vi "Ecrire Prog MODBUS EPC.vi"(0 "Adresse rég":u8 caption="Adresse régulateur", 1 "Programme":cluster{"chaîne o":string, "Value":dbl}[][](array[cluster]), 2 "N° prog":u16 caption="Numéro de programme", 3 "error in":errorcluster caption="error IO", 4 "Port COM run 1 REG":refnum<visa-resource-name>) -> (6 "error out":errorcluster caption="error IO")   [LabVIEW 2022 SP3]
uses:
  Variables globales/Variables glob EUROTHERM.vi
panel:
  out "error IO":errorcluster caption="error par segment"
  out "unité rampe":u16
  out "unité palier":u16
  out "Numéro segment":u16
  out "adr type fin":u64
  out "Nom rég":string caption="Nom régulateur"
  # "écrire un programme"
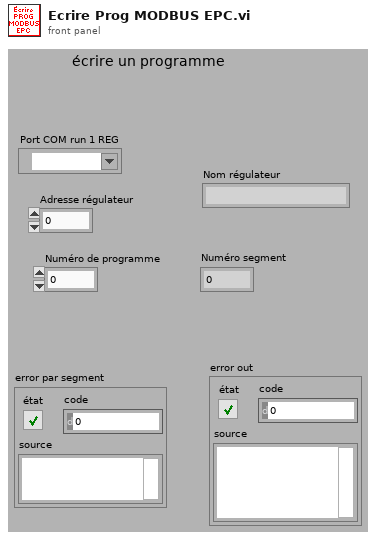
[diagram p1: front panel]
types:
  T1 = typedef "Semaphore RefNum" = refnum<k1>
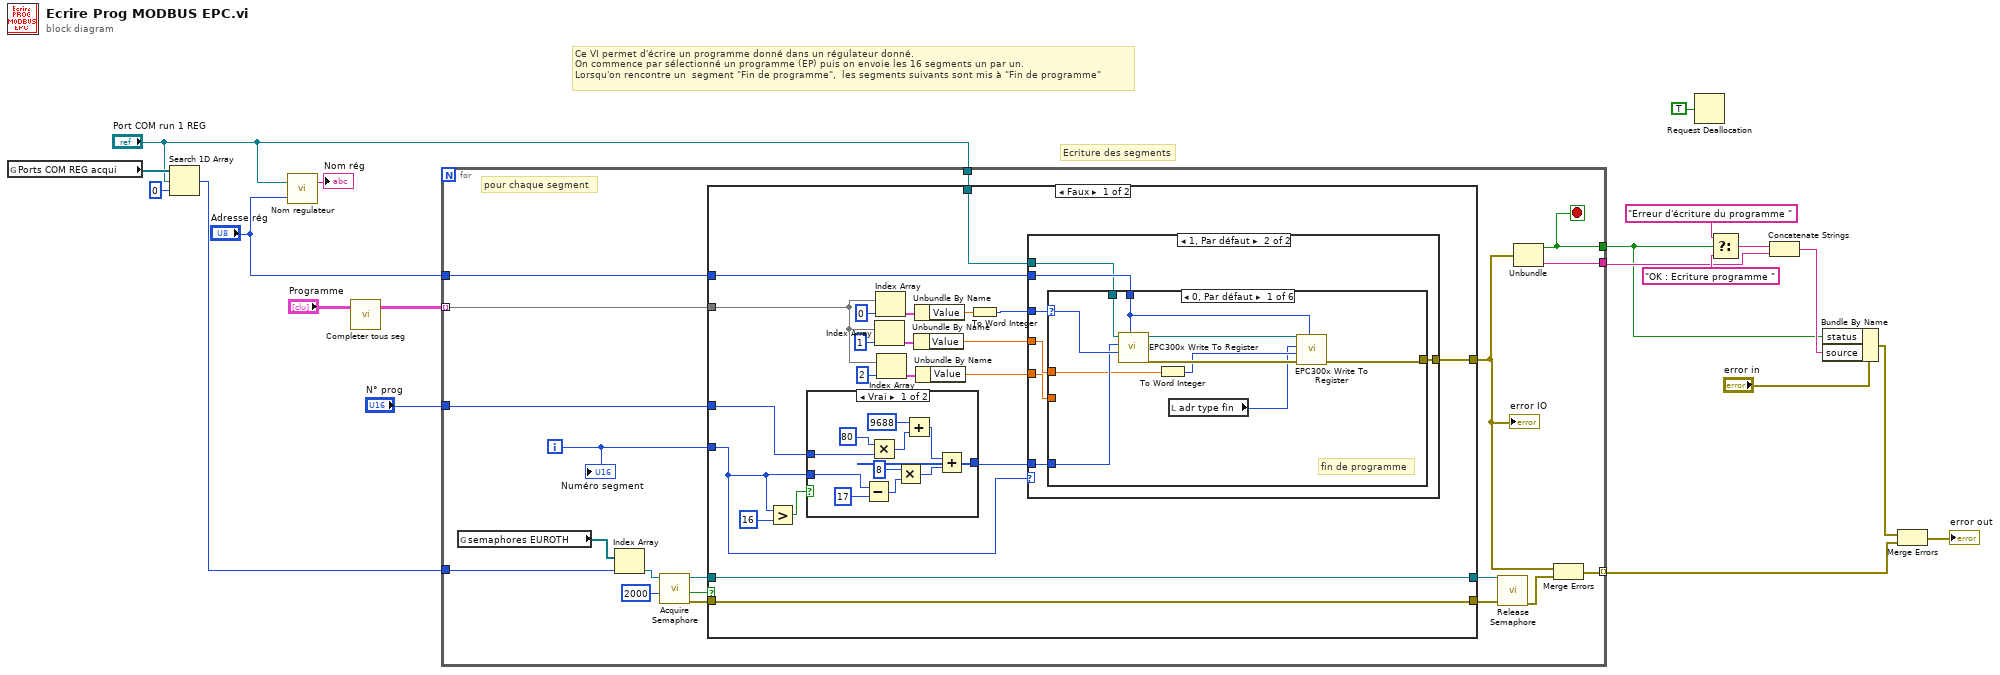
[diagram p0: block diagram]
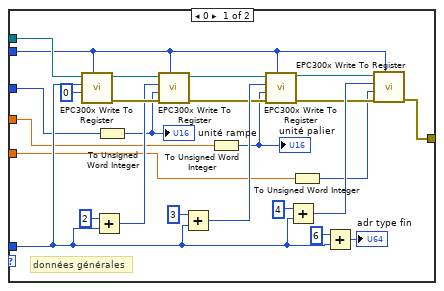
[diagram p2: hidden frame]
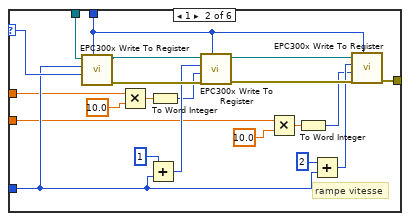
[diagram p3: hidden frame]
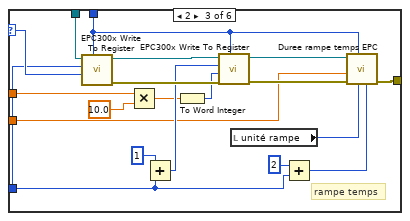
[diagram p4: hidden frame]
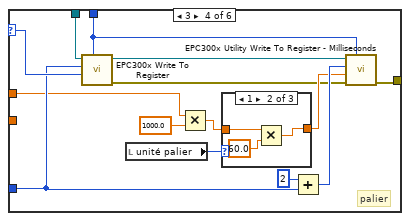
[diagram p5: hidden frame]
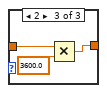
[diagram p7: hidden frame]
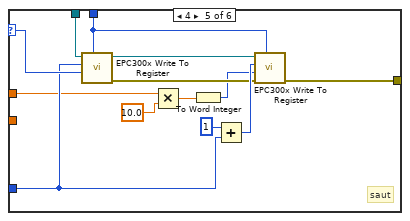
[diagram p8: hidden frame]
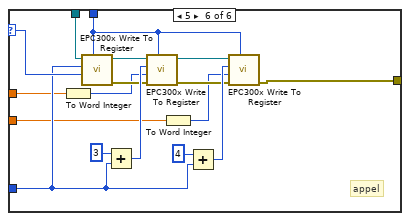
[diagram p9: hidden frame]
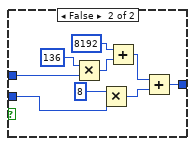
[diagram p10: hidden frame]
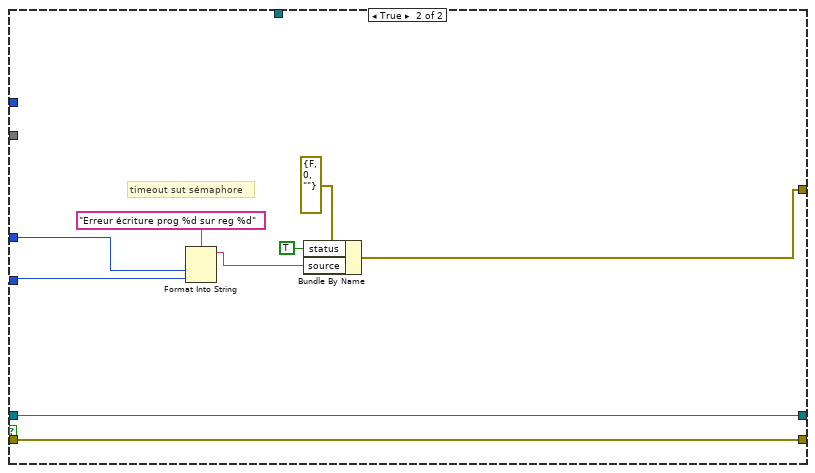
[diagram p11: hidden frame]
diagram:
  # "Ecriture des segments"
  # "Ce VI permet d'écrire un programme donné dans un régulateur donné.\nOn commence par sélectionné un programme (EP) puis on envoie les 16 segments un par un.\nLorsqu'on rencontre un  segment \"Fin de programme\",  les segments suivants sont mis à \"Fin de programme\""
  n1 = global read "Variables glob EUROTHERM.vi" "Ports COM REG acqui"() -> (w14:refnum<visa-resource-name>[])
  n2 = Search 1D Array(1D array=w14, element="Port COM run 1 REG", start index (0)=0 ("indice de départ (0)")) -> (index of element=w11:i32)
  n3 = call "Nom regulateur.vi"("Adresse régulateur"="Adresse rég", "Port COM run 1 REG"="Port COM run 1 REG") -> ("Nom régulateur"=→"Nom rég":string)  [unwired: 1 in]
  n4 = call "Completer tous seg.vi"("Programme"="Programme") -> ("Programme avec tous les segments"=w1:cluster{"chaîne o":string, "Value":dbl}[][])  [unwired: 2 in]
  n5 = for {
    tunnel: w1 -> [w36] mode=indexing
    tunnel: "Port COM run 1 REG" -> [w37]
    tunnel: "N° prog" -> [w39]
    tunnel: "Adresse rég" -> [w35]
    tunnel: [w38] -> w6
    tunnel: w11 -> [w30]
    tunnel: [w21] -> w4
    tunnel: [w22] -> w2 mode=indexing
    i -> [w34]
    stop <- w21 stop-if-true
    # "pour chaque segment"
    n6 = global read "Variables glob EUROTHERM.vi" "semaphores EUROTH"() -> (w32:T1[])
    n7 = Index Array(array=w32, index=w30) -> (element=w33:T1)
    n8 = call <vilib>:"Acquire Semaphore.vi"("ms timeout (-1)"=2000, "semaphore"=w33) -> ("error out"=w27:errorcluster, "timed out"=w29:bool, "semaphore out"=w28:T1)  [unwired: 3 in]
    n9 = case shown="Faux" w29 {
      tunnel: w39 -> [w42 w218]
      tunnel: w37 -> [w58 _]
      tunnel: w36 -> [w53 _]
      tunnel: w35 -> [w51 _]
      tunnel: [w49 w214] -> w23
      tunnel: w34 -> [w41 w217]
      tunnel: [w46 w216] -> w26
      tunnel: w28 -> [w46 w216]
      tunnel: w27 -> [w45 w215]
      tunnel: [w45 w215] -> w25
      frame False {
        n10 = Greater?(x=w41, y=u16 16) -> (0:w44:bool)
        n11 = case shown="Vrai" w44 {
          tunnel: w41 -> [w196 w206]
          tunnel: w42 -> [w195 w207]
          tunnel: [w194 w205] -> w40
          frame True {
            n12 = Subtract(x=w196, y=u16 17) -> (x-y=w197:i32)
            n13 = Multiply(x=u16 80, y=w195) -> (x*y=w201:u16)
            n14 = Multiply(x=u16 8, y=w197) -> (x*y=w203:i32)
            n15 = Add(x=u16 9688, y=w201) -> (x+y=w199:u16)
            n16 = Add(x=w199, y=w203) -> (x+y=w194:i32)
          }
          frame False {
            n17 = Multiply(x=u16 136, y=w207) -> (x*y=w210:u16)
            n18 = Multiply(x=u16 8, y=w206) -> (x*y=w212:i32)
            n19 = Add(x=u16 8192, y=w210) -> (x+y=w208:u16)
            n20 = Add(x=w208, y=w212) -> (x+y=w205:i32)
          }
        }
        n21 = Index Array(array=w53, index=1 ("indice")) -> (element=w57:cluster{"chaîne o":string, "Value":dbl})
        n22 = Index Array(array=w53, index=0 ("indice")) -> (element=w59:cluster{"chaîne o":string, "Value":dbl})
        n23 = Index Array(array=w53, index=2 ("indice")) -> (element=w54:cluster{"chaîne o":string, "Value":dbl})
        n24 = Unbundle By Name(w57) -> ("Value"=w50:dbl)
        n25 = Unbundle By Name(w59) -> ("Value"=w48:dbl)
        n26 = Unbundle By Name(w54) -> ("Value"=w52:dbl)
        n27 = To Word Integer(number=w48) -> (16bit integer=w47:i16)
        n28 = case shown="1, Par défaut" w41 {
          tunnel: w47 -> [w66 w92]
          tunnel: w40 -> [w74 w89]
          tunnel: w58 -> [w76 w90]
          tunnel: w52 -> [w62 w87]
          tunnel: w51 -> [w68 w91]
          tunnel: w50 -> [w63 w88]
          tunnel: [w77 w86] -> w49
          frame 0 {
            # "données générales"
            n29 = call "EPC300x Write To Register.vi"("Unit Address (1)"=w68, "Data (0)"=i16 0, "Register Address (0)"=w74, "VISA session"=w76) -> ("error out"=w70:errorcluster, "dup VISA session"=w72:refnum<visa-resource-name>)  [unwired: 6 in]
            n30 = Add(x=u64 2 ("y"), y=w74) -> (x+y=w67:u64)
            n31 = To Unsigned Word Integer(number=w66) -> (unsigned 16bit integer=w65:u16)
            "unité rampe" <- w65
            n32 = call "EPC300x Write To Register.vi"("Unit Address (1)"=w68, "error in (no error)"=w70, "Data (0)"=w65, "Register Address (0)"=w67, "VISA session"=w72) -> ("error out"=w69:errorcluster, "dup VISA session"=w71:refnum<visa-resource-name>)  [unwired: 5 in]
            n33 = Add(x=u64 3 ("y"), y=w74) -> (x+y=w85:u64)
            n34 = To Unsigned Word Integer(number=w63) -> (unsigned 16bit integer=w64:u16)
            "unité palier" <- w64
            n35 = call "EPC300x Write To Register.vi"("Unit Address (1)"=w68, "error in (no error)"=w69, "Data (0)"=w64, "Register Address (0)"=w85, "VISA session"=w71) -> ("error out"=w79:errorcluster, "dup VISA session"=w78:refnum<visa-resource-name>)  [unwired: 5 in]
            n36 = Add(x=u64 4 ("y"), y=w74) -> (x+y=w84:u64)
            n37 = To Unsigned Word Integer(number=w62) -> (unsigned 16bit integer=w61:u16)
            n38 = Add(x=u64 6 ("y"), y=w74) -> (x+y=→"adr type fin":u64)
            n39 = call "EPC300x Write To Register.vi"("Unit Address (1)"=w68, "error in (no error)"=w79, "Data (0)"=w61, "Register Address (0)"=w84, "VISA session"=w78) -> ("error out"=w77:errorcluster)  [unwired: 5 in, 1 out]
          }
          frame 1, Default {
            n40 = case shown="0, Par défaut" w92 {
              selector: w92 -> [w101 w123 w142 w156 w176 w193]
              tunnel: w91 -> [w99 w119 w131 w148 w174 w181]
              tunnel: w90 -> [w102 w118 w138 w154 w173 w191]
              tunnel: w89 -> [w96 w120 w139 w153 w168 w182]
              tunnel: w88 -> [w95 w110 w134 w151 w167 w180]
              tunnel: w87 -> [_ w109 w127 _ _ w178]
              tunnel: [w97 w111 w128 w143 w169 w183] -> w86
              frame 0, Default {
                # "fin de programme"
                n41 = call "EPC300x Write To Register.vi"("Unit Address (1)"=w99, "Data (0)"=w101, "Register Address (0)"=w96, "VISA session"=w102) -> ("error out"=w98:errorcluster, "dup VISA session"=w100:refnum<visa-resource-name>)  [unwired: 6 in]
                n42 = To Word Integer(number=w95) -> (16bit integer=w94:i16)
                n43 = local read "adr type fin"() -> (w93:u64)
                n44 = call "EPC300x Write To Register.vi"("Unit Address (1)"=w99, "error in (no error)"=w98, "Data (0)"=w94, "Register Address (0)"=w93, "VISA session"=w100) -> ("error out"=w97:errorcluster)  [unwired: 5 in, 1 out]
              }
              frame 1 {
                # "rampe vitesse"
                n45 = call "EPC300x Write To Register.vi"("Unit Address (1)"=w119, "Data (0)"=w123, "Register Address (0)"=w120, "VISA session"=w118) -> ("error out"=w117:errorcluster, "dup VISA session"=w113:refnum<visa-resource-name>)  [unwired: 6 in]
                n46 = Multiply(x=w110, y=10.0 ("cas faux")) -> (x*y=w106:dbl)
                n47 = Add(x=u64 1 ("y"), y=w120) -> (x+y=w115:u64)
                n48 = To Word Integer(number=w106) -> (16bit integer=w105:i16)
                n49 = call "EPC300x Write To Register.vi"("Unit Address (1)"=w119, "error in (no error)"=w117, "Data (0)"=w105, "Register Address (0)"=w115, "VISA session"=w113) -> ("error out"=w116:errorcluster, "dup VISA session"=w112:refnum<visa-resource-name>)  [unwired: 5 in]
                n50 = Multiply(x=w109, y=10.0 ("cas faux")) -> (x*y=w108:dbl)
                n51 = To Word Integer(number=w108) -> (16bit integer=w107:i16)
                n52 = Add(x=u64 2 ("y"), y=w120) -> (x+y=w114:u64)
                n53 = call "EPC300x Write To Register.vi"("Unit Address (1)"=w119, "error in (no error)"=w116, "Data (0)"=w107, "Register Address (0)"=w114, "VISA session"=w112) -> ("error out"=w111:errorcluster)  [unwired: 5 in, 1 out]
              }
              frame 2 {
                # "rampe temps"
                n54 = call "EPC300x Write To Register.vi"("Unit Address (1)"=w131, "Data (0)"=w142, "Register Address (0)"=w139, "VISA session"=w138) -> ("error out"=w137:errorcluster, "dup VISA session"=w135:refnum<visa-resource-name>)  [unwired: 6 in]
                n55 = Multiply(x=w134, y=10.0 ("cas faux")) -> (x*y=w133:dbl)
                n56 = Add(x=u16 1 ("y"), y=w139) -> (x+y=w136:i32)
                n57 = To Word Integer(number=w133) -> (16bit integer=w132:i16)
                n58 = call "EPC300x Write To Register.vi"("Unit Address (1)"=w131, "error in (no error)"=w137, "Data (0)"=w132, "Register Address (0)"=w136, "VISA session"=w135) -> ("error out"=w129:errorcluster, "dup VISA session"=w130:refnum<visa-resource-name>)  [unwired: 5 in]
                n59 = local read "unité rampe"() -> (w126:u16)
                n60 = Add(x=u64 2 ("y"), y=w139) -> (x+y=w125:u64)
                n61 = call "Duree rampe temps EPC.vi"("Registre Address"=w125, "Unité rampe"=w126, "Unit Address (1)"=w131, "entrée d'erreur (pas d'erreur)"=w129, "Durée"=w127, "Refnum VISA en entrée"=w130) -> ("sortie d'erreur"=w128:errorcluster)  [unwired: 4 in, 1 out]
              }
              frame 3 {
                # "palier"
                n62 = call "EPC300x Write To Register.vi"("Unit Address (1)"=w148, "Data (0)"=w156, "Register Address (0)"=w153, "VISA session"=w154) -> ("error out"=w144:errorcluster, "dup VISA session"=w147:refnum<visa-resource-name>)  [unwired: 6 in]
                n63 = local read "unité palier"() -> (w150:u16)
                n64 = Multiply(x=w151, y=1000.0 ("cas faux")) -> (x*y=w149:dbl)
                n65 = case shown="1" w150 {
                  tunnel: w149 -> [w157 w159 w162]
                  tunnel: [w157 w160 w163] -> w145
                  frame 0, Default {
                  }
                  frame 1 {
                    n66 = Multiply(x=w159, y=60.0) -> (x*y=w160:dbl)
                  }
                  frame 2 {
                    n67 = Multiply(x=w162, y=3600.0) -> (x*y=w163:dbl)
                  }
                }
                n68 = Add(x=u64 2 ("y"), y=w153) -> (x+y=w146:u64)
                n69 = call "EPC300x Utility Write To Register - Milliseconds.vi"("Unit Address (1)"=w148, "error in (no error)"=w144, "Data in ms (0)"=w145, "Register Address (0)"=w146, "VISA session"=w147) -> ("error out"=w143:errorcluster)  [unwired: 5 in, 1 out]
              }
              frame 4 {
                # "saut"
                n70 = call "EPC300x Write To Register.vi"("Unit Address (1)"=w174, "Data (0)"=w176, "Register Address (0)"=w168, "VISA session"=w173) -> ("error out"=w171:errorcluster, "dup VISA session"=w170:refnum<visa-resource-name>)  [unwired: 6 in]
                n71 = Multiply(x=w167, y=10.0 ("cas faux")) -> (x*y=w166:dbl)
                n72 = To Word Integer(number=w166) -> (16bit integer=w165:i16)
                n73 = Add(x=u64 1 ("y"), y=w168) -> (x+y=w172:u64)
                n74 = call "EPC300x Write To Register.vi"("Unit Address (1)"=w174, "error in (no error)"=w171, "Data (0)"=w165, "Register Address (0)"=w172, "VISA session"=w170) -> ("error out"=w169:errorcluster)  [unwired: 5 in, 1 out]
              }
              frame 5 {
                # "appel"
                n75 = To Word Integer(number=w180) -> (16bit integer=w179:i16)
                n76 = call "EPC300x Write To Register.vi"("Unit Address (1)"=w181, "Data (0)"=w193, "Register Address (0)"=w182, "VISA session"=w191) -> ("error out"=w187:errorcluster, "dup VISA session"=w185:refnum<visa-resource-name>)  [unwired: 6 in]
                n77 = Add(x=u16 3 ("y"), y=w182) -> (x+y=w189:i32)
                n78 = call "EPC300x Write To Register.vi"("Unit Address (1)"=w181, "error in (no error)"=w187, "Data (0)"=w179, "Register Address (0)"=w189, "VISA session"=w185) -> ("error out"=w186:errorcluster, "dup VISA session"=w184:refnum<visa-resource-name>)  [unwired: 5 in]
                n79 = To Word Integer(number=w178) -> (16bit integer=w177:i16)
                n80 = Add(x=u16 4 ("y"), y=w182) -> (x+y=w190:i32)
                n81 = call "EPC300x Write To Register.vi"("Unit Address (1)"=w181, "error in (no error)"=w186, "Data (0)"=w177, "Register Address (0)"=w190, "VISA session"=w184) -> ("error out"=w183:errorcluster)  [unwired: 5 in, 1 out]
              }
            }
          }
        }
      }
      frame True {
        # "timeout sut sémaphore"
        n82 = Format Into String(format string="Erreur écriture prog %d sur reg %d" ("chaîne de format"), w218, w217) -> (resulting string=w222:string)  [unwired: 2 in, 1 out]
        n83 = Bundle By Name(cluster=errorcluster {"status"=FALSE, "code"=0, "source"=""} ("error IO"), "status"=TRUE, "source"=w222) -> (w214:errorcluster)
      }
    }
    "error IO" <- w23
    n84 = call <vilib>:"Release Semaphore.vi"("error in (no error)"=w25, "semaphore"=w26) -> ("error out"=w24:errorcluster)  [unwired: 4 in, 1 out]
    n85 = Unbundle(w23) -> ("status"=w21:bool, "source"=w38:string)  [unwired: 1 out]
    n86 = Merge Errors(w23, w24) -> (w22:errorcluster)
    "Numéro segment" <- w34
  }
  n87 = Request Deallocation(TRUE ("flag")) -> ()
  n88 = Select(t="Erreur d'écriture du programme ", s=w4, f="OK : Ecriture programme ") -> (s? t:f=w8:string)
  n89 = Concatenate Strings(w8, w6) -> (w7:string)
  n90 = Bundle By Name(cluster="error in", "status"=w4, "source"=w7) -> (w3:errorcluster)
  n91 = Merge Errors(w3, w2) -> (→"error out":errorcluster)
